vi "Stop Core.vi"(10 "final error code":i32, 11 "Actor in":refnum<class "CounterActor.lvclass">) -> (3 "Actor out":refnum<class "CounterActor.lvclass">)   [LabVIEW 2026, in "CounterActor.lvclass"]
doc: "Message Counter actor method: Stop Core. Counter and Processed are private actor state."
uses:
  CounterActor.lvclass
  <vilib>/ActorFramework/Actor/Actor.lvclass
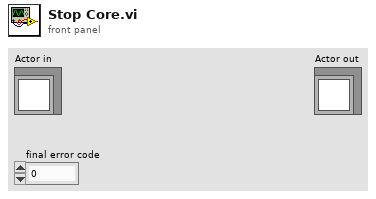
[diagram p1: front panel]
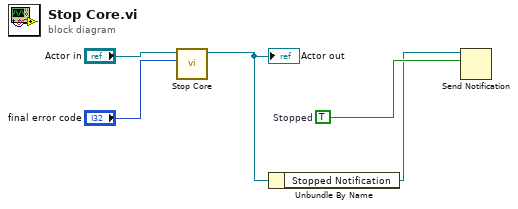
[diagram p0: block diagram]
diagram:
  w5 = TRUE  # Stopped
  n1 = call-parent "Stop Core.vi"("final error code"="final error code", "Actor in"="Actor in") -> ("Actor out"=w3:refnum<class "CounterActor.lvclass">)  [unwired: 9 in]
  "Actor out" <- w3
  n2 = Unbundle By Name(w3) -> ("Stopped Notification"=w4:refnum<notifier>)
  n3 = Send Notification(notification=w5, notifier=w4) -> ()  [unwired: 1 in, 2 out]
